vi "ReadAIOData.vi"(8 "error in (no error)":errorcluster, 11 "object in":refnum<class "AIO-Configuration.lvclass">) -> (0 "error out":errorcluster, 2 "Data":T1, 3 "object out":refnum<class "AIO-Configuration.lvclass">)   [LabVIEW 2021, in "AIO-Channel.lvlib" / "AIO-Configuration.lvclass"]
uses:
  AIO-Configuration.lvclass
  tdef/Data.ctl
  tdef/Direction.ctl
  AIO-Configuration.lvclass/AIO-Configuration.ctl
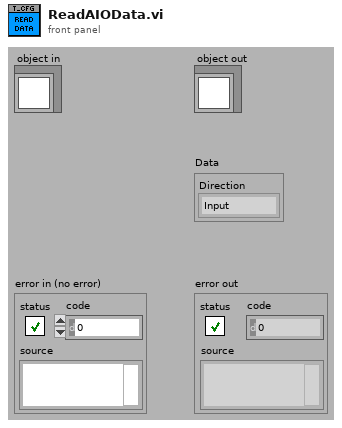
[diagram p1: front panel]
types:
  T1 = typedef "AIO-Channel.lvlib/AIO-Configuration.lvclass/Data.ctl" = cluster{"Direction":T2}
  T2 = typedef "AIO-Channel.lvlib/AIO-Configuration.lvclass/Direction.ctl" = enum16{"Input", "Output"}
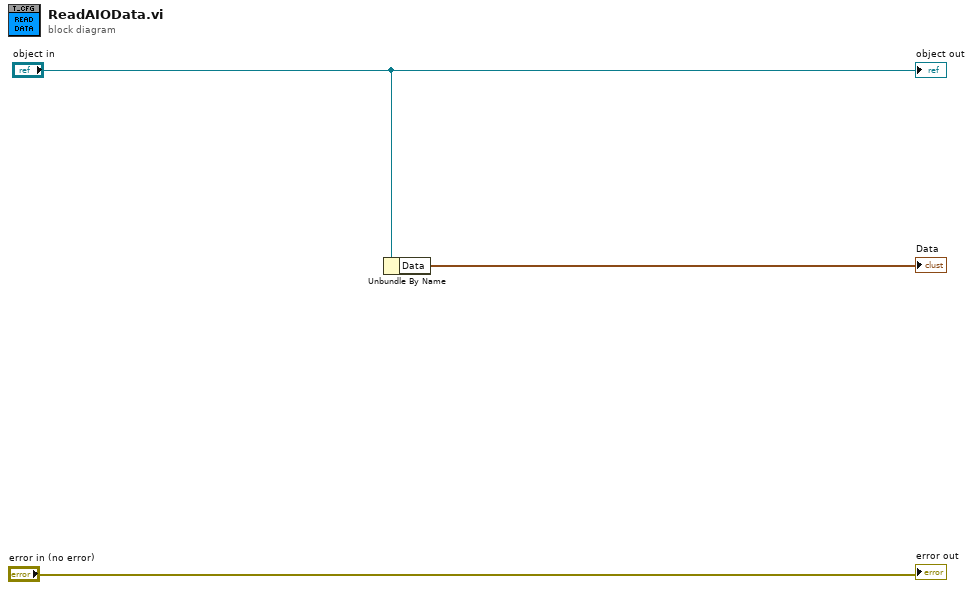
[diagram p0: block diagram]
diagram:
  n1 = Unbundle By Name("object in") -> ("Data"=→"Data":T1)
  "error out" <- "error in (no error)"
  "object out" <- "object in"
